vi "Valve Picture.vi"(7 "Valve Pictures":T3, 10 "Unused Element":T2, 11 "Values":T7) -> (1 "Energized Picture":T1, 2 "Feedback Picture":T1, 3 "Command Picture":T1)   [LabVIEW 2020, in "VolatusGUIElements.lvlib" / "2WayValveV.lvclass"]
uses:
  2WayValveV.lvclass
  Values.ctl
  Channel State.ctl
  Valve Pictures.ctl
  Command Pictures.ctl
  Picture.ctl
  Feedback Pictures.ctl
  Energized Pictures.ctl
  Unused Element.ctl
  Picture.vi
  2WayValveV.lvclass/2WayValveV.ctl
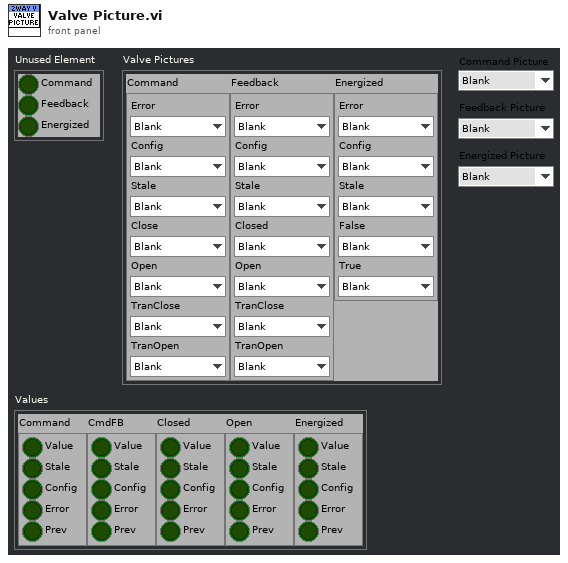
[diagram p1: front panel]
types:
  T1 = typedef "VolatusGUIElements.lvlib/2WayValveV.lvclass/Picture.ctl" = enum16{"Blank", "OutClose", "OutOpen", "OutTranClose", "OutTranOpen", "OutConfig", "OutStale", "OutError", "InClose", "InOpen", "InTranClose", "InTranOpen", "InConfig", "InStale", "InError", "EnOff", "EnOn", "EnConfig", "EnStale", "EnError"}
  T2 = typedef "VolatusGUIElements.lvlib/2WayValveV.lvclass/Unused Element.ctl" = cluster{"Command":bool, "Feedback":bool, "Energized":bool}
  T3 = typedef "VolatusGUIElements.lvlib/2WayValveV.lvclass/Valve Pictures.ctl" = cluster{"Command":T4, "Feedback":T5, "Energized":T6}
  T4 = typedef "VolatusGUIElements.lvlib/2WayValveV.lvclass/Command Pictures.ctl" = cluster{"Error":T1, "Config":T1, "Stale":T1, "Close":T1, "Open":T1, "TranClose":T1, "TranOpen":T1}
  T5 = typedef "VolatusGUIElements.lvlib/2WayValveV.lvclass/Feedback Pictures.ctl" = cluster{"Error":T1, "Config":T1, "Stale":T1, "Closed":T1, "Open":T1, "TranClose":T1, "TranOpen":T1}
  T6 = typedef "VolatusGUIElements.lvlib/2WayValveV.lvclass/Energized Pictures.ctl" = cluster{"Error":T1, "Config":T1, "Stale":T1, "False":T1, "True":T1}
  T7 = typedef "VolatusGUIElements.lvlib/2WayValveV.lvclass/Values.ctl" = cluster{"Command":T8, "CmdFB":T8, "Closed":T8, "Open":T8, "Energized":T8}
  T8 = typedef "VolatusGUIElements.lvlib/2WayValveV.lvclass/Channel State.ctl" = cluster{"Value":bool, "Stale":bool, "Config":bool, "Error":bool, "Prev":bool}
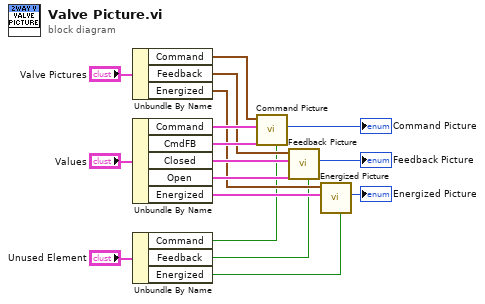
[diagram p0: block diagram]
diagram:
  n1 = Unbundle By Name("Valve Pictures") -> ("Command"=w15:T4, "Feedback"=w11:T5, "Energized"=w8:T6)
  n2 = Unbundle By Name("Values") -> ("Command"=w14:T8, "CmdFB"=w13:T8, "Closed"=w12:T8, "Open"=w10:T8, "Energized"=w9:T8)
  n3 = Unbundle By Name("Unused Element") -> ("Command"=w4:bool, "Feedback"=w5:bool, "Energized"=w6:bool)
  n4 = call "Command Picture.vi"("Unused"=w4, "Feedback State"=w13, "Command State"=w14, "Command Pictures"=w15) -> ("Command Picture"=→"Command Picture":T1)  [unwired: 7 in]
  n5 = call "Feedback Picture.vi"("Unused"=w5, "Open State"=w10, "Closed State"=w12, "Feedback Pictures"=w11) -> ("Feedback Picture"=→"Feedback Picture":T1)  [unwired: 7 in]
  n6 = call "Energized Picture.vi"("Unused"=w6, "Energized State"=w9, "Energized Pictures"=w8) -> ("Energized Picture"=→"Energized Picture":T1)  [unwired: 8 in]
